vi "Test_Queue.vi"() -> (2 "Tests":cluster{"Test":string, "Passed":bool}[](array[cluster]), 3 "All Passed":bool)   [LabVIEW 2021]
uses:
  fb02bb9d-60fe-4efe-999d-8fafea34c26a.vi
  86eb2c31-2ef4-4f52-8c7e-c4cd79eee94b.vi
  15bb192a-e047-4910-b6c7-e2d91b4fb920.vi
  07afb981-15fc-4acc-97a8-0c99b9836663.vi
  0269a72d-fd89-4c26-9187-e43185b182b9.vi
  803f4470-47be-4643-a591-48d54bf1cc4c.vi
  7d11f8f4-9aa5-40e4-88f9-cf15113ac809.vi
  3fbf7aaa-d5ae-4bec-ab0e-4ac27ad070b2.vi
  1ab1bd47-603c-456c-b9d0-96944e88f92c.vi
  ebbe48c1-b72b-4de3-aeb3-ba80bb7d0d19.vi
  8bdc6467-f6e5-4f75-9ac6-95094b1edd2b.vi
  fafea8c6-e71b-47bf-8fdc-74539dc463ec.vi
  be416df7-4f26-4020-a28b-5e551047e503.vi
  6a558a1d-279f-4cd8-a1d4-0ce029900aa4.vi
  7b643780-0266-49a5-bff5-7ddf02e75eca.vi
  src/Queue.lvlib
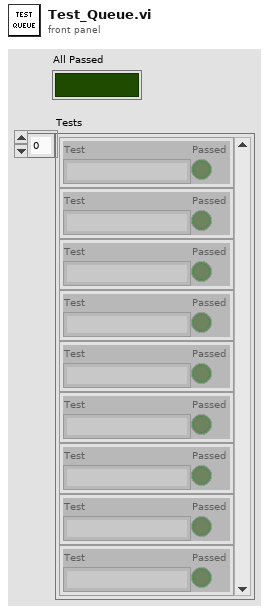
[diagram p1: front panel]
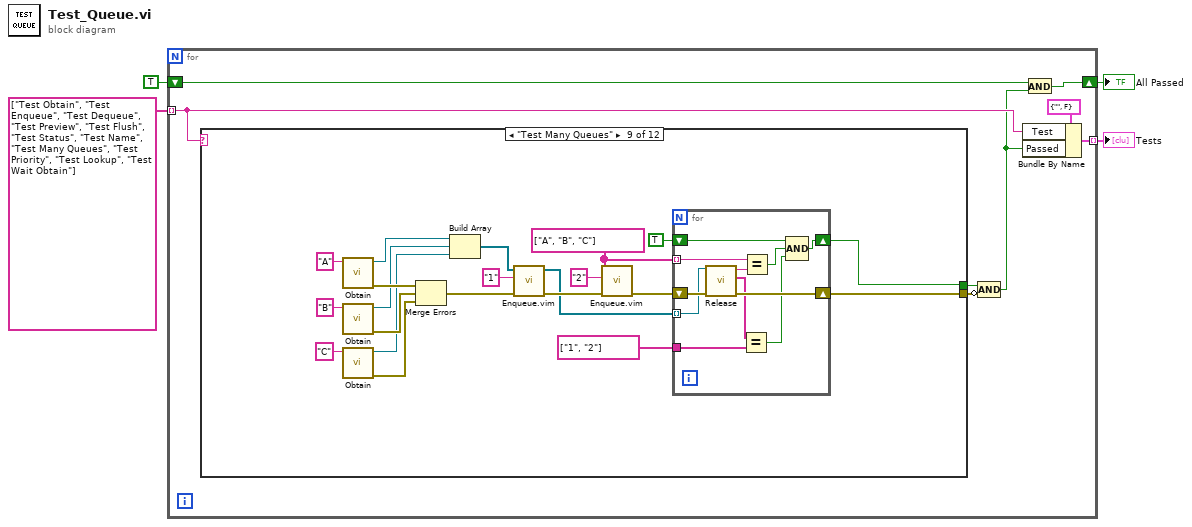
[diagram p0: block diagram]
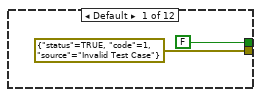
[diagram p2: hidden frame]
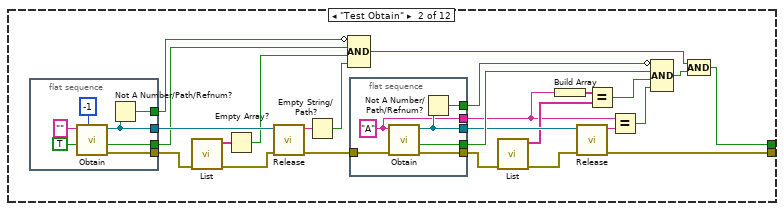
[diagram p3: hidden frame]
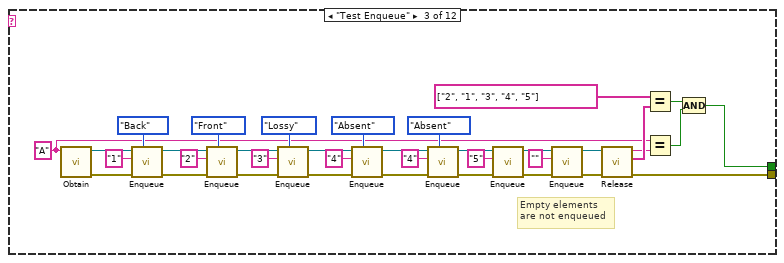
[diagram p4: hidden frame]
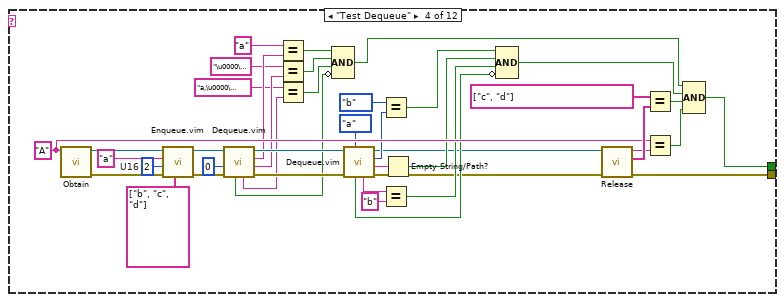
[diagram p5: hidden frame]
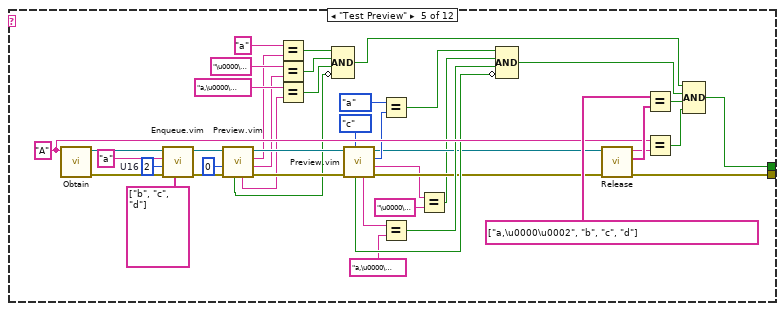
[diagram p6: hidden frame]
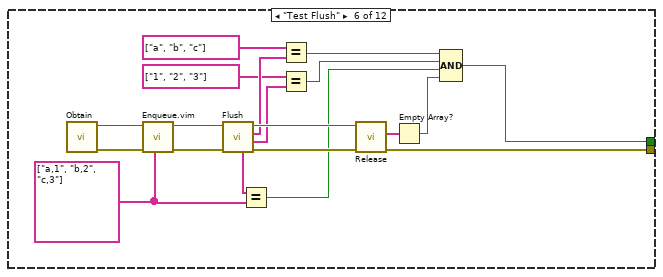
[diagram p7: hidden frame]
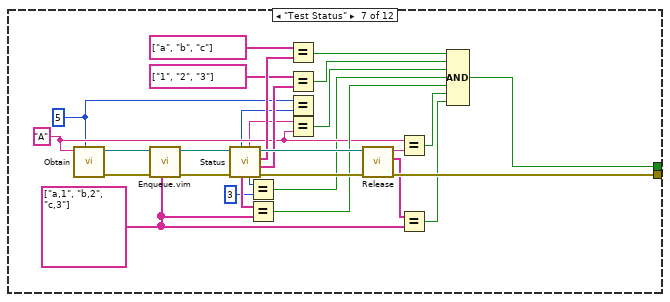
[diagram p8: hidden frame]
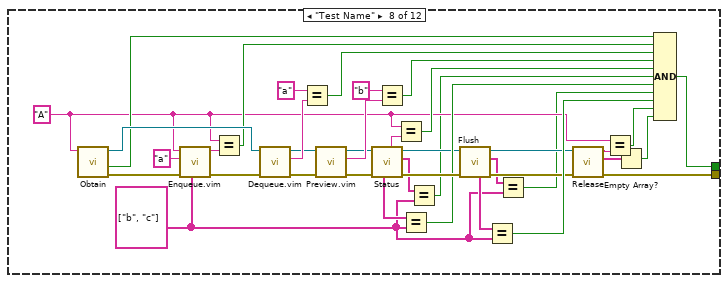
[diagram p9: hidden frame]
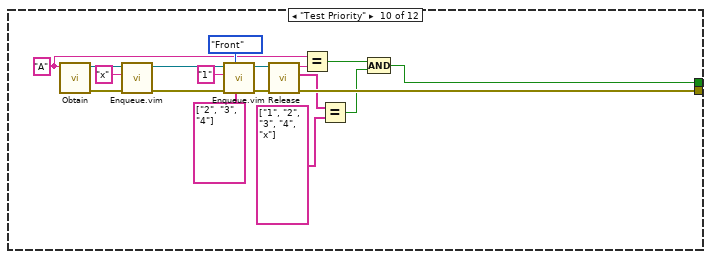
[diagram p10: hidden frame]
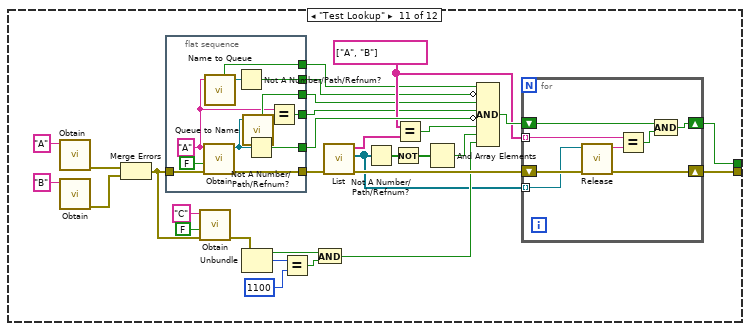
[diagram p11: hidden frame]
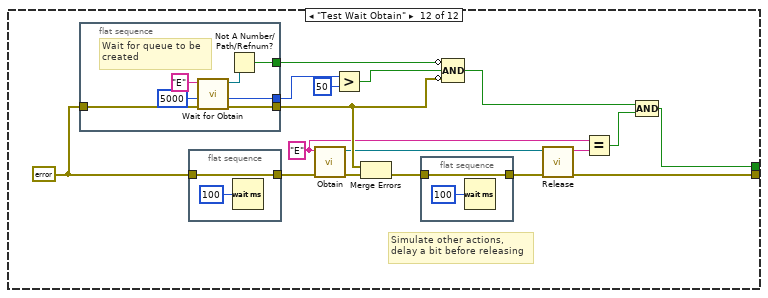
[diagram p12: hidden frame]
diagram:
  n1 = for {
    tunnel: string[] ["Test Obtain", "Test Enqueue", "Test Dequeue", "Test Preview", "Test Flush", "Test Status", "Test Name", "Test Many Queues", "Test Priority", "Test Lookup", "Test Wait Obtain"] -> [w8] mode=indexing
    shift-right: [w10] -> w2
    shift-left: TRUE -> [w11]
    tunnel: [w9] -> w1 mode=indexing
    n2 = case shown="\"Test Many Queues\"" w8 {
      tunnel: [FALSE w30 w64 w126 w169 w180 w213 w231 w262 w298 w338 w366] -> w7
      tunnel: [errorcluster {"status"=TRUE, "code"=1, "source"="Invalid Test Case"} ("error in (no error)") w29 w67 w129 w172 w192 w221 w232 w266 w305 w340 w371] -> w5
      frame Default {
      }
      frame "Test Obtain" {
        n3 = flat-sequence {
          tunnel: [w52] -> w24
          tunnel: [w50] -> w39
          tunnel: [w49] -> w38
          tunnel: [w48] -> w37
          frame #0 {
            n4 = call "Obtain.vi"("Max Size (-1=Unlimited)"=-1, "Create if not Found? (T)"=TRUE, "Queue Name (\"\"=Unnamed)"="" ("Queue Name (\"\"=Unnamed)")) -> ("error out"=w52:errorcluster, "Created New?"=w48:bool, "Queue out"=w50:refnum<queue>)  [unwired: 6 in]
            n5 = Not A Number/Path/Refnum?(number/path/refnum=w50) -> (NaN/Path/Refnum?=w49:bool)
          }
        }
        n6 = call "List.vi"("error in (no error)"=w24) -> ("error out"=w23:errorcluster, "Queue Names"=w22:string[])  [unwired: 8 in, 1 out]
        n7 = Empty Array?(array=w22) -> (empty?=w21:bool)
        n8 = call "Release.vi"("error in (no error)"=w23, "Queue in"=w39) -> ("error out"=w33:errorcluster, "Queue Name"=w26:string)  [unwired: 7 in, 1 out]
        n9 = Empty String/Path?(string/path=w26) -> (empty?=w25:bool)
        n10 = Compound Arithmetic op=AND(invert w38, w37, w21, w25) -> (w31:bool)
        n11 = flat-sequence {
          tunnel: [w45] -> w36
          tunnel: [w44] -> w35
          tunnel: [w43] -> w34
          tunnel: [w42] -> w20
          tunnel: w33 -> [w41]
          tunnel: [w40] -> w16
          frame #0 {
            w40 = "A" ("Queue Name (\"\"=Unnamed)")
            n12 = call "Obtain.vi"("error in (no error)"=w41, "Queue Name (\"\"=Unnamed)"=w40) -> ("error out"=w42:errorcluster, "Created New?"=w45:bool, "Queue out"=w43:refnum<queue>)  [unwired: 7 in]
            n13 = Not A Number/Path/Refnum?(number/path/refnum=w43) -> (NaN/Path/Refnum?=w44:bool)
          }
        }
        n14 = call "List.vi"("error in (no error)"=w20) -> ("error out"=w19:errorcluster, "Queue Names"=w18:string[])  [unwired: 8 in, 1 out]
        n15 = Build Array(w16) -> (w17:string[])
        n16 = call "Release.vi"("error in (no error)"=w19, "Queue in"=w34) -> ("error out"=w29:errorcluster, "Queue Name"=w28:string)  [unwired: 7 in, 1 out]
        n17 = Equal?(x=w17, y=w18) -> (x = y?=w15:bool)
        n18 = Equal?(x=w16, y=w28) -> (x = y?=w27:bool)
        n19 = Compound Arithmetic op=AND(invert w35, w36, w15, w27) -> (w32:bool)
        n20 = Compound Arithmetic op=AND(w31, w32) -> (w30:bool)
      }
      frame "Test Enqueue" {
        w61 = "A" ("Queue Name (\"\"=Unnamed)")
        # "Empty elements\nare not enqueued"
        n21 = call "Obtain.vi"("Queue Name (\"\"=Unnamed)"=w61) -> ("error out"=w87:errorcluster, "Queue out"=w88:refnum<queue>)  [unwired: 8 in, 1 out]
        n22 = call "Enqueue.vi"("Method (Back)"=enum8{"Back", "Front", "Lossy", "Absent"}."Back", "error in (no error)"=w87, "Element"="1", "Queue in"=w88) -> ("error out"=w81:errorcluster, "Queue out"=w82:refnum<queue>)  [unwired: 6 in]
        n23 = call "Enqueue.vi"("Method (Back)"=enum8{"Back", "Front", "Lossy", "Absent"}."Front", "error in (no error)"=w81, "Element"="2", "Queue in"=w82) -> ("error out"=w77:errorcluster, "Queue out"=w78:refnum<queue>)  [unwired: 6 in]
        n24 = call "Enqueue.vi"("Method (Back)"=enum8{"Back", "Front", "Lossy", "Absent"}."Lossy", "error in (no error)"=w77, "Element"="3", "Queue in"=w78) -> ("error out"=w73:errorcluster, "Queue out"=w74:refnum<queue>)  [unwired: 6 in]
        n25 = call "Enqueue.vi"("Method (Back)"=enum8{"Back", "Front", "Lossy", "Absent"}."Absent", "error in (no error)"=w73, "Element"="4", "Queue in"=w74) -> ("error out"=w69:errorcluster, "Queue out"=w70:refnum<queue>)  [unwired: 6 in]
        n26 = call "Enqueue.vi"("Method (Back)"=enum8{"Back", "Front", "Lossy", "Absent"}."Absent", "error in (no error)"=w69, "Element"="4", "Queue in"=w70) -> ("error out"=w59:errorcluster, "Queue out"=w60:refnum<queue>)  [unwired: 6 in]
        n27 = call "Enqueue.vi"("error in (no error)"=w59, "Element"="5", "Queue in"=w60) -> ("error out"=w56:errorcluster, "Queue out"=w57:refnum<queue>)  [unwired: 7 in]
        n28 = call "Enqueue.vi"("error in (no error)"=w56, "Element"="", "Queue in"=w57) -> ("error out"=w55:errorcluster, "Queue out"=w54:refnum<queue>)  [unwired: 7 in]
        n29 = call "Release.vi"("error in (no error)"=w55, "Queue in"=w54) -> ("error out"=w67:errorcluster, "Remaining Elements"=w66:string[], "Queue Name"=w63:string)  [unwired: 7 in]
        n30 = Equal?(x=string[] ["2", "1", "3", "4", "5"] ("y"), y=w66) -> (x = y?=w65:bool)
        n31 = Equal?(x=w61, y=w63) -> (x = y?=w62:bool)
        n32 = Compound Arithmetic op=AND(w65, w62) -> (w64:bool)
      }
      frame "Test Dequeue" {
        w119 = u16 2  # U16
        w123 = "A" ("Queue Name (\"\"=Unnamed)")
        n33 = call "Obtain.vi"("Queue Name (\"\"=Unnamed)"=w123) -> ("error out"=w121:errorcluster, "Queue out"=w122:refnum<queue>)  [unwired: 8 in, 1 out]
        n34 = call "Enqueue.vim"("Messages"=string[] ["b", "c", "d"], "error in (no error)"=w121, "Data"=w119, "Message"="a", "Queue in"=w122) -> ("error out"=w117:errorcluster, "Queue out"=w116:refnum<queue>)  [unwired: 5 in]
        n35 = call "Dequeue.vim"("error in (no error)"=w117, "Timeout in ms (-1)"=0, "Queue in"=w116) -> ("error out"=w114:errorcluster, "Data"=w110:string, "Message"=w112:string, "Queue out"=w113:refnum<queue>, "Element"=w105:string, "Timed Out?"=w103:bool)  [unwired: 3 in]
        n36 = Equal?(x="a", y=w112) -> (x = y?=w108:bool)
        n37 = Equal?(x="\u0000\u0002", y=w110) -> (x = y?=w107:bool)
        n38 = Equal?(x="a,\u0000\u0002", y=w105) -> (x = y?=w104:bool)
        n39 = Compound Arithmetic op=AND(w108, w107, w104, invert w103) -> (w89:bool)
        n40 = call "Dequeue.vim"("Message Type"=enum16{"a", "b", "c", "d"}."a", "error in (no error)"=w114, "Queue in"=w113) -> ("error out"=w92:errorcluster, "Data"=w98:string, "Message"=w101:enum16{"a", "b", "c", "d"}, "Queue out"=w91:refnum<queue>, "Element"=w96:string, "Timed Out?"=w93:bool)  [unwired: 3 in]
        n41 = Equal?(x=enum16{"a", "b", "c", "d"}."b", y=w101) -> (x = y?=w99:bool)
        n42 = Equal?(x=w96, y="b") -> (x = y?=w94:bool)
        n43 = Empty String/Path?(string/path=w98) -> (empty?=w97:bool)
        n44 = Compound Arithmetic op=AND(w99, w97, w94, invert w93) -> (w90:bool)
        n45 = call "Release.vi"("error in (no error)"=w92, "Queue in"=w91) -> ("error out"=w129:errorcluster, "Remaining Elements"=w128:string[], "Queue Name"=w125:string)  [unwired: 7 in]
        n46 = Equal?(x=string[] ["c", "d"] ("y"), y=w128) -> (x = y?=w127:bool)
        n47 = Equal?(x=w123, y=w125) -> (x = y?=w124:bool)
        n48 = Compound Arithmetic op=AND(w89, w90, w127, w124) -> (w126:bool)
      }
      frame "Test Preview" {
        w162 = u16 2  # U16
        w166 = "A" ("Queue Name (\"\"=Unnamed)")
        n49 = call "Obtain.vi"("Queue Name (\"\"=Unnamed)"=w166) -> ("error out"=w164:errorcluster, "Queue out"=w165:refnum<queue>)  [unwired: 8 in, 1 out]
        n50 = call "Enqueue.vim"("Messages"=string[] ["b", "c", "d"], "error in (no error)"=w164, "Data"=w162, "Message"="a", "Queue in"=w165) -> ("error out"=w143:errorcluster, "Queue out"=w142:refnum<queue>)  [unwired: 5 in]
        n51 = call "Preview.vim"("error in (no error)"=w143, "Timeout in ms (-1)"=0, "Queue in"=w142) -> ("error out"=w140:errorcluster, "Data"=w136:string, "Message"=w135:string, "Queue out"=w141:refnum<queue>, "Element"=w138:string, "Timed Out?"=w137:bool)  [unwired: 3 in]
        n52 = Equal?(x="a", y=w135) -> (x = y?=w158:bool)
        n53 = Equal?(x="\u0000\u0002", y=w136) -> (x = y?=w157:bool)
        n54 = Equal?(x="a,\u0000\u0002", y=w138) -> (x = y?=w155:bool)
        n55 = Compound Arithmetic op=AND(w158, w157, w155, invert w137) -> (w144:bool)
        n56 = call "Preview.vim"("Message Type"=enum16{"a", "b", "c", "d"}."c", "error in (no error)"=w140, "Queue in"=w141) -> ("error out"=w147:errorcluster, "Data"=w132:string, "Message"=w153:enum16{"a", "b", "c", "d"}, "Queue out"=w146:refnum<queue>, "Element"=w150:string, "Timed Out?"=w148:bool)  [unwired: 3 in]
        n57 = Equal?(x=enum16{"a", "b", "c", "d"}."a", y=w153) -> (x = y?=w151:bool)
        n58 = Equal?(x=w150, y="a,\u0000\u0002" ("x")) -> (x = y?=w149:bool)
        n59 = Equal?(x=w132, y="\u0000\u0002" ("x")) -> (x = y?=w131:bool)
        n60 = Compound Arithmetic op=AND(w151, w131, w149, invert w148) -> (w145:bool)
        n61 = call "Release.vi"("error in (no error)"=w147, "Queue in"=w146) -> ("error out"=w172:errorcluster, "Remaining Elements"=w171:string[], "Queue Name"=w168:string)  [unwired: 7 in]
        n62 = Equal?(x=string[] ["a,\u0000\u0002", "b", "c", "d"] ("y"), y=w171) -> (x = y?=w170:bool)
        n63 = Equal?(x=w166, y=w168) -> (x = y?=w167:bool)
        n64 = Compound Arithmetic op=AND(w144, w145, w170, w167) -> (w169:bool)
      }
      frame "Test Flush" {
        w184 = string[] ["a,1", "b,2", "c,3"] ("Messages")
        n65 = call "Obtain.vi"() -> ("error out"=w188:errorcluster, "Queue out"=w189:refnum<queue>)  [unwired: 9 in, 1 out]
        n66 = call "Enqueue.vim"("Messages"=w184, "error in (no error)"=w188, "Queue in"=w189) -> ("error out"=w186:errorcluster, "Queue out"=w187:refnum<queue>)  [unwired: 7 in]
        n67 = call "Flush.vi"("error in (no error)"=w186, "Queue in"=w187) -> ("error out"=w191:errorcluster, "Data"=w176:string[], "Messages"=w179:string[], "Queue out"=w190:refnum<queue>, "Elements"=w185:string[])  [unwired: 5 in]
        n68 = Equal?(x=w185, y=w184) -> (x = y?=w181:bool)
        n69 = Equal?(x=string[] ["a", "b", "c"], y=w179) -> (x = y?=w174:bool)
        n70 = Equal?(x=string[] ["1", "2", "3"], y=w176) -> (x = y?=w175:bool)
        n71 = call "Release.vi"("error in (no error)"=w191, "Queue in"=w190) -> ("error out"=w192:errorcluster, "Remaining Elements"=w183:string[])  [unwired: 7 in, 1 out]
        n72 = Empty Array?(array=w183) -> (empty?=w182:bool)
        n73 = Compound Arithmetic op=AND(w174, w175, w181, w182) -> (w180:bool)
      }
      frame "Test Status" {
        w197 = 5 ("Max Size (-1=Unlimited)")
        w201 = "A" ("Queue Name (\"\"=Unnamed)")
        w204 = string[] ["a,1", "b,2", "c,3"] ("Messages")
        n74 = call "Obtain.vi"("Max Size (-1=Unlimited)"=w197, "Queue Name (\"\"=Unnamed)"=w201) -> ("error out"=w217:errorcluster, "Queue out"=w218:refnum<queue>)  [unwired: 7 in, 1 out]
        n75 = call "Enqueue.vim"("Messages"=w204, "error in (no error)"=w217, "Queue in"=w218) -> ("error out"=w215:errorcluster, "Queue out"=w216:refnum<queue>)  [unwired: 7 in]
        n76 = call "Status.vi"("error in (no error)"=w215, "Queue in"=w216) -> ("error out"=w220:errorcluster, "Data"=w209:string[], "Messages"=w212:string[], "Queue out"=w219:refnum<queue>, "# Elements in Queue"=w196:i32, "Queue Name"=w200:string, "Elements"=w206:string[], "Max Size"=w198:i32)  [unwired: 2 in]
        n77 = Equal?(x=w196, y=3) -> (x = y?=w194:bool)
        n78 = Equal?(x=w206, y=w204) -> (x = y?=w214:bool)
        n79 = Equal?(x=string[] ["a", "b", "c"], y=w212) -> (x = y?=w207:bool)
        n80 = Equal?(x=string[] ["1", "2", "3"], y=w209) -> (x = y?=w208:bool)
        n81 = Equal?(x=w197, y=w198) -> ()  [unwired: 1 out]
        n82 = Equal?(x=w200, y=w201) -> (x = y?=w199:bool)
        n83 = call "Release.vi"("error in (no error)"=w220, "Queue in"=w219) -> ("error out"=w221:errorcluster, "Remaining Elements"=w205:string[], "Queue Name"=w202:string)  [unwired: 7 in]
        n84 = Equal?(x=w201, y=w202) -> (x = y?=w193:bool)
        n85 = Equal?(x=w205, y=w204) -> (x = y?=w203:bool)
        n86 = Compound Arithmetic op=AND(w207, w208, w199, w194, w214, w193, w203) -> (w213:bool)
      }
      frame "Test Name" {
        w223 = string[] ["b", "c"] ("Messages")
        w236 = "A" ("Queue Name (\"\"=Unnamed)")
        n87 = call "Obtain.vi"("Queue Name (\"\"=Unnamed)"=w236) -> ("error out"=w260:errorcluster, "Created New?"=w253:bool, "Queue out"=w257:refnum<queue>)  [unwired: 8 in]
        n88 = call "Enqueue.vim"("Messages"=w223, "error in (no error)"=w260, "Message"="a", "Queue in"=w236) -> ("error out"=w258:errorcluster, "Queue out"=w245:string)  [unwired: 6 in]
        n89 = Equal?(x=w236, y=w245) -> (x = y?=w244:bool)
        n90 = call "Dequeue.vim"("error in (no error)"=w258, "Queue in"=w257) -> ("error out"=w252:errorcluster, "Message"=w256:string, "Queue out"=w251:refnum<queue>)  [unwired: 4 in, 3 out]
        n91 = Equal?(x="a", y=w256) -> (x = y?=w254:bool)
        n92 = call "Preview.vim"("error in (no error)"=w252, "Queue in"=w251) -> ("error out"=w247:errorcluster, "Message"=w249:string, "Queue out"=w230:refnum<queue>)  [unwired: 4 in, 3 out]
        n93 = call "Status.vi"("error in (no error)"=w247, "Queue in"=w230) -> ("error out"=w246:errorcluster, "Messages"=w224:string[], "Queue out"=w229:refnum<queue>, "Queue Name"=w228:string, "Elements"=w243:string[])  [unwired: 2 in, 3 out]
        n94 = Equal?(x="b", y=w249) -> (x = y?=w248:bool)
        n95 = Equal?(x=w236, y=w228) -> (x = y?=w242:bool)
        n96 = Equal?(x=w243, y=w223) -> (x = y?=w241:bool)
        n97 = Equal?(x=w224, y=w223) -> (x = y?=w222:bool)
        n98 = call "Flush.vi"("error in (no error)"=w246, "Queue in"=w229) -> ("error out"=w238:errorcluster, "Messages"=w226:string[], "Queue out"=w227:refnum<queue>, "Elements"=w240:string[])  [unwired: 5 in, 1 out]
        n99 = Equal?(x=w240, y=w223) -> (x = y?=w239:bool)
        n100 = Equal?(x=w226, y=w223) -> (x = y?=w225:bool)
        n101 = call "Release.vi"("error in (no error)"=w238, "Queue in"=w227) -> ("error out"=w232:errorcluster, "Remaining Elements"=w234:string[], "Queue Name"=w237:string)  [unwired: 7 in]
        n102 = Equal?(x=w236, y=w237) -> (x = y?=w235:bool)
        n103 = Empty Array?(array=w234) -> (empty?=w233:bool)
        n104 = Compound Arithmetic op=AND(w253, w244, w254, w248, w242, w222, w241, w225, w239, w235, w233) -> (w231:bool)
      }
      frame "Test Many Queues" {
        w265 = string[] ["A", "B", "C"]
        n105 = call "Obtain.vi"("Queue Name (\"\"=Unnamed)"="A" ("Queue Name (\"\"=Unnamed)")) -> ("error out"=w278:errorcluster, "Queue out"=w271:refnum<queue>)  [unwired: 8 in, 1 out]
        n106 = call "Obtain.vi"("Queue Name (\"\"=Unnamed)"="B" ("Queue Name (\"\"=Unnamed)")) -> ("error out"=w279:errorcluster, "Queue out"=w270:refnum<queue>)  [unwired: 8 in, 1 out]
        n107 = call "Obtain.vi"("Queue Name (\"\"=Unnamed)"="C" ("Queue Name (\"\"=Unnamed)")) -> ("error out"=w276:errorcluster, "Queue out"=w269:refnum<queue>)  [unwired: 8 in, 1 out]
        n108 = Merge Errors(w278, w279, w276) -> (w273:errorcluster)
        n109 = Build Array(w271, w270, w269) -> (w268:refnum<queue>[])
        n110 = call "Enqueue.vim"("error in (no error)"=w273, "Message"="1", "Queue in"=w268) -> ("error out"=w272:errorcluster, "Queue out"=w261:refnum<queue>[])  [unwired: 7 in]
        n111 = call "Enqueue.vim"("error in (no error)"=w272, "Message"="2", "Queue in"=w265) -> ("error out"=w267:errorcluster)  [unwired: 7 in, 1 out]
        n112 = for {
          shift-right: [w291] -> w266
          shift-left: w267 -> [w292]
          tunnel: w265 -> [w289] mode=indexing
          tunnel: string[] ["1", "2"] ("y") -> [w287]
          shift-right: [w284] -> w262
          shift-left: TRUE -> [w283]
          tunnel: w261 -> [w282] mode=indexing
          n113 = call "Release.vi"("error in (no error)"=w292, "Queue in"=w282) -> ("error out"=w291:errorcluster, "Remaining Elements"=w288:string[], "Queue Name"=w290:string)  [unwired: 7 in]
          n114 = Equal?(x=w288, y=w287) -> (x = y?=w285:bool)
          n115 = Equal?(x=w289, y=w290) -> (x = y?=w286:bool)
          n116 = Compound Arithmetic op=AND(w283, w286, w285) -> (w284:bool)
        }
      }
      frame "Test Priority" {
        w302 = "A" ("Queue Name (\"\"=Unnamed)")
        n117 = call "Obtain.vi"("Queue Name (\"\"=Unnamed)"=w302) -> ("error out"=w296:errorcluster, "Queue out"=w297:refnum<queue>)  [unwired: 8 in, 1 out]
        n118 = call "Enqueue.vim"("error in (no error)"=w296, "Message"="x", "Queue in"=w297) -> ("error out"=w295:errorcluster, "Queue out"=w294:refnum<queue>)  [unwired: 7 in]
        n119 = call "Enqueue.vim"("Messages"=string[] ["2", "3", "4"], "Method (Back)"=enum8{"Back", "Front", "Lossy", "Absent"}."Front", "error in (no error)"=w295, "Message"="1", "Queue in"=w294) -> ("error out"=w307:errorcluster, "Queue out"=w306:refnum<queue>)  [unwired: 5 in]
        n120 = call "Release.vi"("error in (no error)"=w307, "Queue in"=w306) -> ("error out"=w305:errorcluster, "Remaining Elements"=w304:string[], "Queue Name"=w303:string)  [unwired: 7 in]
        n121 = Equal?(x=w302, y=w303) -> (x = y?=w300:bool)
        n122 = Equal?(x=w304, y=string[] ["1", "2", "3", "4", "x"]) -> (x = y?=w299:bool)
        n123 = Compound Arithmetic op=AND(w300, w299) -> (w298:bool)
      }
      frame "Test Lookup" {
        w316 = string[] ["A", "B"] ("y")
        n124 = call "Obtain.vi"("Queue Name (\"\"=Unnamed)"="A" ("Queue Name (\"\"=Unnamed)")) -> ("error out"=w337:errorcluster)  [unwired: 8 in, 2 out]
        n125 = call "Obtain.vi"("Queue Name (\"\"=Unnamed)"="B" ("Queue Name (\"\"=Unnamed)")) -> ("error out"=w335:errorcluster)  [unwired: 8 in, 2 out]
        n126 = Merge Errors(w337, w335) -> (w332:errorcluster)
        n127 = flat-sequence {
          tunnel: w332 -> [w359]
          tunnel: [w358] -> w326
          tunnel: [w357] -> w325
          tunnel: [w355] -> w315
          tunnel: [w354] -> w314
          tunnel: [w352] -> w313
          tunnel: [w349] -> w312
          frame #0 {
            w350 = "A" ("Queue Name (\"\"=Unnamed)")
            n128 = call "Obtain.vi"("error in (no error)"=w359, "Create if not Found? (T)"=FALSE, "Queue Name (\"\"=Unnamed)"=w350) -> ("error out"=w357:errorcluster, "Queue out"=w353:refnum<queue>)  [unwired: 6 in, 1 out]
            n129 = call "Name to Queue.vi"("Queue Name in"=w350) -> ("Found?"=w354:bool, "Queue out"=w356:refnum<queue>)  [unwired: 7 in]
            n130 = Not A Number/Path/Refnum?(number/path/refnum=w356) -> (NaN/Path/Refnum?=w355:bool)
            n131 = call "Queue to Name.vi"("Queue in"=w353) -> ("Found?"=w352:bool, "Queue Name out"=w351:string)  [unwired: 7 in]
            n132 = Not A Number/Path/Refnum?(number/path/refnum=w353) -> (NaN/Path/Refnum?=w358:bool)
            n133 = Equal?(x=w350, y=w351) -> (x = y?=w349:bool)
          }
        }
        n134 = call "Obtain.vi"("error in (no error)"=w332, "Create if not Found? (T)"=FALSE, "Queue Name (\"\"=Unnamed)"="C" ("Queue Name (\"\"=Unnamed)")) -> ("error out"=w331:errorcluster)  [unwired: 6 in, 2 out]
        n135 = Unbundle(w331) -> ("status"=w329:bool, "code"=w330:i32)  [unwired: 1 out]
        n136 = Equal?(x=w330, y=1100) -> (x = y?=w328:bool)
        n137 = And(x=w329, y=w328) -> (x .and. y?=w322:bool)
        n138 = call "List.vi"("error in (no error)"=w325) -> ("error out"=w323:errorcluster, "Queues"=w311:refnum<queue>[], "Queue Names"=w321:string[])  [unwired: 8 in]
        n139 = Not A Number/Path/Refnum?(number/path/refnum=w311) -> (NaN/Path/Refnum?=w320:bool[])
        n140 = Not(x=w320) -> (.not. x?=w319:bool[])
        n141 = Equal?(x=w316, y=w321) -> (x = y?=w324:bool)
        n142 = And Array Elements(Boolean array=w319) -> (logical AND=w318:bool)
        n143 = Compound Arithmetic op=AND(w314, invert w315, w313, w312, invert w326, w324, w318, w322) -> (w317:bool)
        n144 = for {
          shift-right: [w348] -> w340
          shift-left: w323 -> [w344]
          shift-right: [w345] -> w338
          shift-left: w317 -> [w343]
          tunnel: w316 -> [w342] mode=indexing
          tunnel: w311 -> [w341] mode=indexing
          n145 = call "Release.vi"("error in (no error)"=w344, "Queue in"=w341) -> ("error out"=w348:errorcluster, "Queue Name"=w347:string)  [unwired: 7 in, 1 out]
          n146 = Equal?(x=w342, y=w347) -> (x = y?=w346:bool)
          n147 = Compound Arithmetic op=AND(w343, w346) -> (w345:bool)
        }
      }
      frame "Test Wait Obtain" {
        w377 = errorcluster {"status"=FALSE, "code"=0, "source"=""} ("error in (no error)")
        w369 = "E" ("Queue Name (\"\"=Unnamed)")
        # "Simulate other actions,\ndelay a bit before releasing"
        n148 = flat-sequence {
          tunnel: w377 -> [w385]
          tunnel: [w382] -> w375
          tunnel: [w381] -> w373
          tunnel: [w380] -> w365
          frame #0 {
            # "Wait for queue to be\ncreated"
            n149 = call "Wait for Obtain.vi"("error in (no error)"=w385, "ms Timeout (5000)"=u32 5000 ("Timeout in ms (5000)"), "Queue Name"="E") -> ("error out"=w381:errorcluster, "ms Elapsed"=w380:u32, "Queue out"=w383:refnum<queue>)  [unwired: 6 in]
            n150 = Not A Number/Path/Refnum?(number/path/refnum=w383) -> (NaN/Path/Refnum?=w382:bool)
          }
        }
        n151 = flat-sequence {
          tunnel: w377 -> [w387]
          tunnel: [w387] -> w376
          frame #0 {
            n152 = Wait (ms)(milliseconds to wait=u32 100) -> ()  [unwired: 1 out]
          }
        }
        n153 = call "Obtain.vi"("error in (no error)"=w376, "Queue Name (\"\"=Unnamed)"=w369) -> ("error out"=w374:errorcluster, "Queue out"=w372:refnum<queue>)  [unwired: 7 in, 1 out]
        n154 = Greater?(x=w365, y=u32 50) -> (0:w363:bool)
        n155 = Merge Errors(w373, w374) -> (w362:errorcluster)
        n156 = flat-sequence {
          tunnel: w362 -> [w378]
          tunnel: [w378] -> w361
          frame #0 {
            n157 = Wait (ms)(milliseconds to wait=u32 100) -> ()  [unwired: 1 out]
          }
        }
        n158 = Compound Arithmetic op=AND(invert w375, w363, invert w373) -> (w367:bool)
        n159 = call "Release.vi"("error in (no error)"=w361, "Queue in"=w372) -> ("error out"=w371:errorcluster, "Queue Name"=w370:string)  [unwired: 7 in, 1 out]
        n160 = Equal?(x=w369, y=w370) -> (x = y?=w368:bool)
        n161 = Compound Arithmetic op=AND(w367, w368) -> (w366:bool)
      }
    }
    n162 = Compound Arithmetic op=AND(w7, invert w5) -> (w6:bool)
    n163 = Bundle By Name(cluster=cluster{"Test":string, "Passed":bool} {"Test"="", "Passed"=FALSE} ("Cluster"), "Test"=w8, "Passed"=w6) -> (w9:cluster{"Test":string, "Passed":bool})
    n164 = And(x=w11, y=w6) -> (x .and. y?=w10:bool)
  }
  "All Passed" <- w2
  "Tests" <- w1
